vi "FuncVI_Sub - Format string to format array.vi"(3 "format string":string) -> (0 "# formats":i32, 1 "formats":cluster{"str":string, "format?":bool}[](array[cluster]))   [LabVIEW 2021]
doc: "::: CalcExpress Toolkit :::\nCopyright (c) 2000-2026 Konstantin Shifershteyn. All rights reserved."
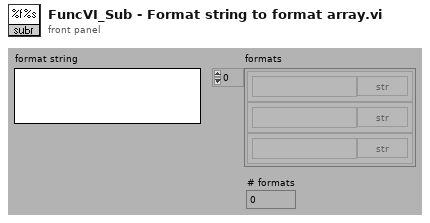
[diagram p1: front panel]
types:
  T1 = cluster{"format string":string, "format specifier":bool}
  T2 = cluster{"format string":string, "format specifier":bool}[]
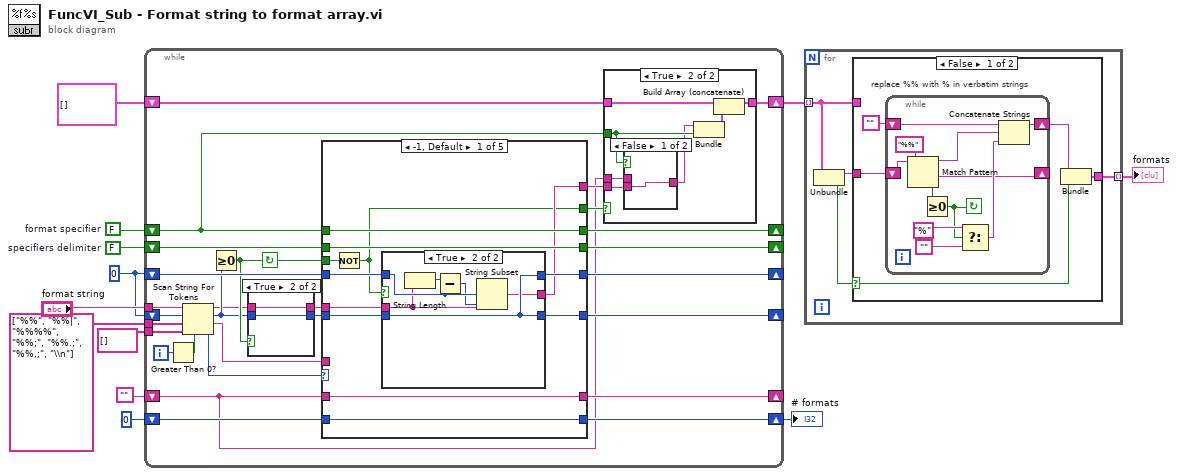
[diagram p0: block diagram]
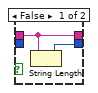
[diagram p2: hidden frame]
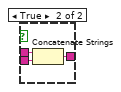
[diagram p4: hidden frame]
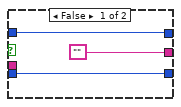
[diagram p5: hidden frame]
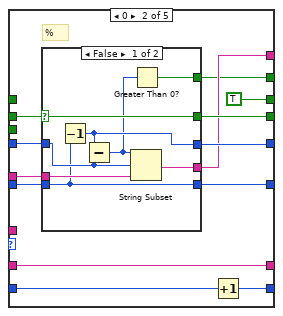
[diagram p6: hidden frame]
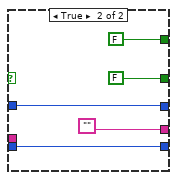
[diagram p7: hidden frame]
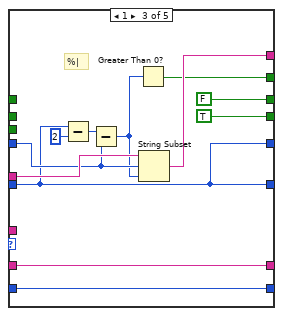
[diagram p8: hidden frame]
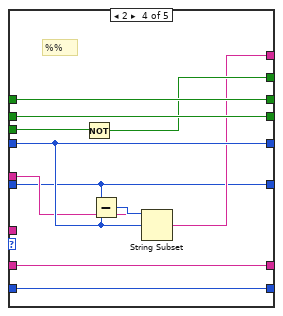
[diagram p9: hidden frame]
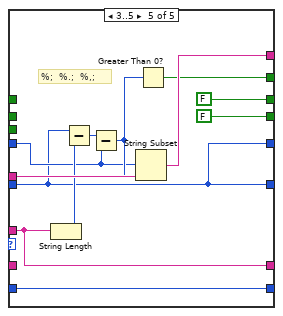
[diagram p10: hidden frame]
diagram:
  w9 = FALSE  # format specifier
  w10 = FALSE  # specifiers delimiter
  w11 = 0 ("offset past token")
  n1 = while {
    shift-left: "" -> [w18]
    shift-right: [w19] -> _
    shift-left: 0 -> [w25]
    shift-right: [w26] -> w5
    tunnel: string[] [] ("delimiters (\\s,\\t,\\r,\\n)") -> [w27]
    shift-left: w9 -> [w22]
    shift-right: [w29] -> _
    shift-left: cluster{"str":string, "format?":bool}[] [] ("formats") -> [w20]
    shift-right: [w23] -> w2
    shift-left: w10 -> [w34]
    shift-right: [w33] -> _
    shift-left: w11 -> [w35]
    shift-right: [w32] -> _
    shift-left: w11 -> [w38]
    shift-right: [w36] -> _
    tunnel: string[] ["%%", "%%|", "%%%%", "%%;", "%%.;", "%%,;", "\\n"] ("operators (none)") -> [w39]
    tunnel: "format string" -> [w40]
    i -> [w37]
    stop <- w17 continue-if-true
    n2 = Greater Than 0?(x=w37) -> (x > 0?=w30:bool)
    n3 = Scan String For Tokens(4:w30, 6:w27, 7:w39, 8:w38, 9:w40) -> (0:w31:i32, 1:w28:string, 2:w15:i32, 3:w14:string)  [unwired: 1 in]
    n4 = Greater Or Equal To 0?(x=w15) -> (x >= 0?=w17:bool)
    n5 = case shown="True" w17 {
      tunnel: [w42 w44] -> w16
      tunnel: w15 -> [_ w44]
      tunnel: w14 -> [w41 w43]
      tunnel: [w41 w43] -> w13
      frame False {
        n6 = String Length(string=w41) -> (length=w42:i32)
      }
      frame True {
      }
    }
    n7 = case shown="-1, Default" w31 {
      tunnel: w16 -> [w68 w88 w111 w116 w128]
      tunnel: [w64 w87 w111 w116 w128] -> w36
      tunnel: w35 -> [w66 w85 w114 w119 w129]
      tunnel: w13 -> [w67 w84 w115 w117 w137]
      tunnel: w34 -> [w63 w90 _ w126 _]
      tunnel: [w63 w86 TRUE w126 FALSE] -> w33
      tunnel: [w65 w89 w111 w119 w128] -> w32
      tunnel: w17 -> [w58 _ _ w122 _]
      tunnel: w22 -> [w62 _ _ w125 _]
      tunnel: [w62 TRUE FALSE w125 FALSE] -> w29
      tunnel: w28 -> [_ _ _ _ w134]
      tunnel: [w61 w83 w108 w124 w135] -> w26
      tunnel: w25 -> [w61 w82 w108 w124 w135]
      tunnel: [w60 w81 w107 w123 w134] -> w19
      tunnel: w18 -> [w60 w81 w107 w123 _]
      tunnel: [w57 w78 w105 w121 w127] -> w24
      tunnel: [w59 w80 w106 w118 w133] -> w21
      frame -1, Default {
        n8 = Not(x=w58) -> (.not. x?=w57:bool)
        n9 = case shown="True" w57 {
          tunnel: [w71 w73] -> w65
          tunnel: w68 -> [w70 w73]
          tunnel: [w70 w73] -> w64
          tunnel: w66 -> [w71 w77]
          tunnel: w67 -> [_ w74]
          tunnel: ["" w72] -> w59
          frame False {
          }
          frame True {
            n10 = String Length(string=w74) -> (length=w75:i32)
            n11 = Subtract(x=w75, y=w77) -> (x-y=w76:i32)
            n12 = String Subset(string=w74, offset (0)=w77, length (rest)=w76) -> (substring=w72:string)
          }
        }
      }
      frame 0 {
        # "%"
        n13 = case shown="False" w90 {
          selector: w90 -> [w98 _]
          tunnel: [w94 w102] -> w89
          tunnel: w88 -> [w95 w101]
          tunnel: [w95 w101] -> w87
          tunnel: [w98 FALSE] -> w86
          tunnel: w85 -> [w96 w102]
          tunnel: w84 -> [w97 _]
          tunnel: [w93 ""] -> w80
          tunnel: [w92 FALSE] -> w78
          frame False {
            n14 = Decrement(x=w95) -> (x-1=w94:i32)
            n15 = Subtract(x=w94, y=w96) -> (x-y=w91:i32)
            n16 = String Subset(string=w97, offset (0)=w96, length (rest)=w91) -> (substring=w93:string)
            n17 = Greater Than 0?(x=w91) -> (x > 0?=w92:bool)
          }
          frame True {
          }
        }
        n18 = Increment(x=w82) -> (x+1=w83:i32)
      }
      frame 1 {
        # "%|"
        n19 = Subtract(x=w111, y=2) -> (x-y=w112:i32)
        n20 = Subtract(x=w112, y=w114) -> (x-y=w104:i32)
        n21 = Greater Than 0?(x=w104) -> (x > 0?=w105:bool)
        n22 = String Subset(string=w115, offset (0)=w114, length (rest)=w104) -> (substring=w106:string)
      }
      frame 2 {
        # "%%"
        n23 = Not(x=w122) -> (.not. x?=w121:bool)
        n24 = Subtract(x=w116, y=w119) -> (x-y=w120:i32)
        n25 = String Subset(string=w117, offset (0)=w119, length (rest)=w120) -> (substring=w118:string)
      }
      frame 3..5 {
        # "%;  %.;  %,;"
        n26 = String Length(string=w134) -> (length=w132:i32)
        n27 = Subtract(x=w128, y=w132) -> (x-y=w131:i32)
        n28 = Subtract(x=w131, y=w129) -> (x-y=w130:i32)
        n29 = String Subset(string=w137, offset (0)=w129, length (rest)=w130) -> (substring=w133:string)
        n30 = Greater Than 0?(x=w130) -> (x > 0?=w127:bool)
      }
    }
    n31 = case shown="True" w24 {
      tunnel: [w45 w52] -> w23
      tunnel: w20 -> [w45 w51]
      tunnel: w22 -> [_ w49]
      tunnel: w18 -> [_ w48]
      tunnel: w21 -> [_ w47]
      frame False {
      }
      frame True {
        n32 = case shown="False" w49 {
          tunnel: w48 -> [_ w56]
          tunnel: w47 -> [w53 w55]
          tunnel: [w53 w54] -> w46
          frame False {
          }
          frame True {
            n33 = Concatenate Strings(w56, w55) -> (w54:string)
          }
        }
        n34 = Bundle("format string"=w46, "format specifier"=w49) -> (w50:T1)  [unwired: 1 in]
        n35 = Build Array (concatenate)(w51, w50) -> (w52:T2)
      }
    }
  }
  "# formats" <- w5
  n36 = for {
    tunnel: w2 -> [w140] mode=indexing
    tunnel: [w139] -> w1 mode=indexing
    n37 = Unbundle(w140) -> ("str"=w141:string, "format?"=w142:bool)
    n38 = case shown="False" w142 {
      selector: w142 -> [w145 _]
      tunnel: w141 -> [w143 _]
      tunnel: w140 -> [_ w159]
      tunnel: [w144 w159] -> w139
      frame False {
        # "replace %% with % in verbatim strings"
        n39 = while {
          shift-left: w143 -> [w149]
          shift-right: [w148] -> _
          shift-left: "" -> [w153]
          shift-right: [w152] -> w146
          stop <- w151 continue-if-true
          n40 = Match Pattern(string=w149, regular expression="%%") -> (before substring=w154:string, after substring=w148:string, offset past match=w150:i32)  [unwired: 1 in, 1 out]
          n41 = Greater Or Equal To 0?(x=w150) -> (x >= 0?=w151:bool)
          n42 = Select(t="%", s=w151, f="") -> (s? t:f=w155:string)
          n43 = Concatenate Strings(w153, w154, w155) -> (w152:string)
        }
        n44 = Bundle(w146, w145) -> (w144:cluster{string, bool})  [unwired: 1 in]
      }
      frame True {
      }
    }
  }
  "formats" <- w1
